vi "Report_path.vi"(8 "error In":errorcluster, 9 "Result":bool) -> (0 "error out":errorcluster, 3 "appended path":path)   [LabVIEW 2021]
panel:
  out "appended path 2":path
  out "path":path
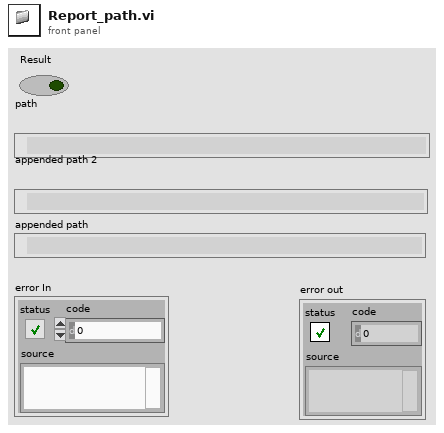
[diagram p1: front panel]
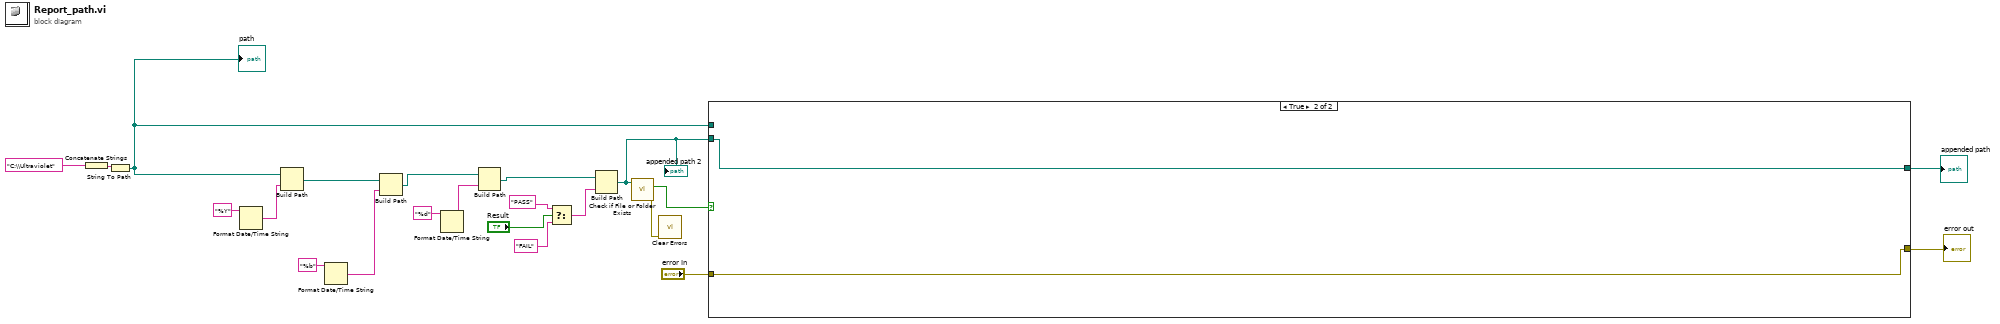
[diagram p0: block diagram]
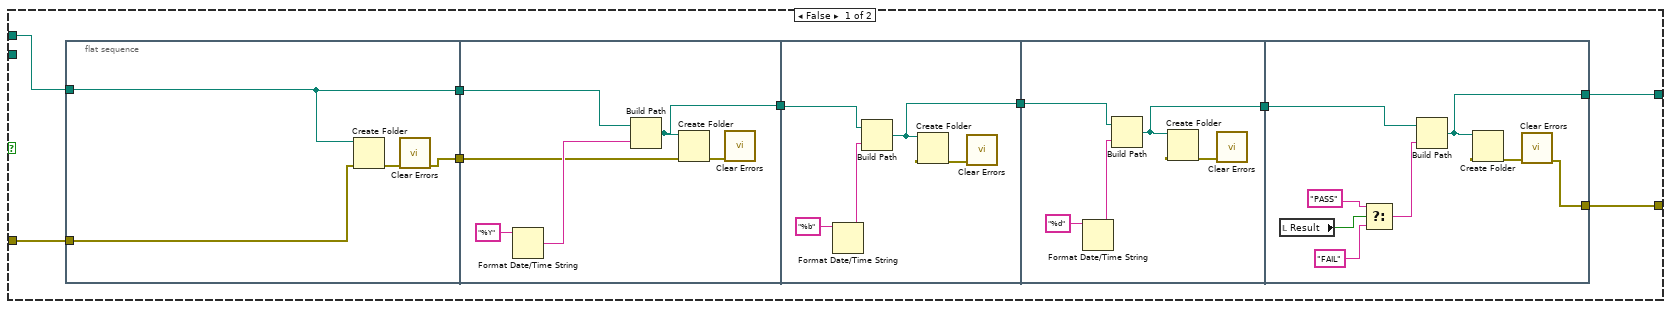
[diagram p2: hidden frame]
diagram:
  n1 = Concatenate Strings("C:\\Ultraviolet" ("string")) -> (w5:string)
  n2 = String To Path(string=w5) -> (path=w3:path)
  "path" <- w3
  n3 = Format Date/Time String(time format string (%c)="%Y") -> (date/time string=w21:string)  [unwired: 2 in]
  n4 = Build Path(base path=w3, name or relative path=w21) -> (appended path=w20:path)
  n5 = Format Date/Time String(time format string (%c)="%b") -> (date/time string=w18:string)  [unwired: 2 in]
  n6 = Build Path(base path=w20, name or relative path=w18) -> (appended path=w15:path)
  n7 = Format Date/Time String(time format string (%c)="%d") -> (date/time string=w17:string)  [unwired: 2 in]
  n8 = Build Path(base path=w15, name or relative path=w17) -> (appended path=w11:path)
  n9 = Select(t="PASS" ("time format string (%c)"), s="Result", f="FAIL" ("time format string (%c)")) -> (s? t:f=w14:string)
  n10 = Build Path(base path=w11, name or relative path=w14) -> (appended path=w8:path)
  "appended path 2" <- w8
  n11 = call <vilib>:"Check if File or Folder Exists.vi"("path"=w8) -> ("error out"=w7:errorcluster, "file or folder exists?"=w6:bool)  [unwired: 8 in, 1 out]
  n12 = call <vilib>:"Clear Errors.vi"("error in (no error)"=w7) -> ()  [unwired: 5 in, 2 out]
  n13 = case shown="True" w6 {
    tunnel: [w27 w61] -> w9
    tunnel: w8 -> [_ w61]
    tunnel: w3 -> [w26 _]
    tunnel: [w25 w60] -> w2
    tunnel: "error In" -> [w24 w60]
    frame False {
      n14 = flat-sequence {
        tunnel: [w34] -> w31
        tunnel: w26 -> [w34]
        tunnel: w24 -> [w33]
        tunnel: [w32] -> w23
        tunnel: [w38] -> w30
        tunnel: w31 -> [w37]
        tunnel: w23 -> [w36]
        tunnel: w30 -> [w44]
        tunnel: [w42] -> w29
        tunnel: w29 -> [w48]
        tunnel: [w47] -> w28
        tunnel: w28 -> [w58]
        tunnel: [w54] -> w27
        tunnel: [w52] -> w25
        frame #0 {
          n15 = Create Folder(path (use dialog)=w34, error in=w33) -> (error out=w35:errorcluster)  [unwired: 1 in, 2 out]
          n16 = call <vilib>:"Clear Errors.vi"("error in (no error)"=w35) -> ("error out"=w32:errorcluster)  [unwired: 5 in, 1 out]
        }
        frame #1 {
          n17 = Format Date/Time String(time format string (%c)="%Y") -> (date/time string=w40:string)  [unwired: 2 in]
          n18 = Build Path(base path=w37, name or relative path=w40) -> (appended path=w38:path)
          n19 = Create Folder(path (use dialog)=w38, error in=w36) -> (error out=w39:errorcluster)  [unwired: 1 in, 2 out]
          n20 = call <vilib>:"Clear Errors.vi"("error in (no error)"=w39) -> ()  [unwired: 5 in, 2 out]
        }
        frame #2 {
          n21 = Format Date/Time String(time format string (%c)="%b") -> (date/time string=w43:string)  [unwired: 2 in]
          n22 = Build Path(base path=w44, name or relative path=w43) -> (appended path=w42:path)
          n23 = Create Folder(path (use dialog)=w42) -> (error out=w46:errorcluster)  [unwired: 2 in, 2 out]
          n24 = call <vilib>:"Clear Errors.vi"("error in (no error)"=w46) -> ()  [unwired: 5 in, 2 out]
        }
        frame #3 {
          n25 = Format Date/Time String(time format string (%c)="%d") -> (date/time string=w51:string)  [unwired: 2 in]
          n26 = Build Path(base path=w48, name or relative path=w51) -> (appended path=w47:path)
          n27 = Create Folder(path (use dialog)=w47) -> (error out=w49:errorcluster)  [unwired: 2 in, 2 out]
          n28 = call <vilib>:"Clear Errors.vi"("error in (no error)"=w49) -> ()  [unwired: 5 in, 2 out]
        }
        frame #4 {
          n29 = local read "Result"() -> (w53:bool)
          n30 = Select(t="PASS" ("time format string (%c)"), s=w53, f="FAIL" ("time format string (%c)")) -> (s? t:f=w55:string)
          n31 = Build Path(base path=w58, name or relative path=w55) -> (appended path=w54:path)
          n32 = Create Folder(path (use dialog)=w54) -> (error out=w59:errorcluster)  [unwired: 2 in, 2 out]
          n33 = call <vilib>:"Clear Errors.vi"("error in (no error)"=w59) -> ("error out"=w52:errorcluster)  [unwired: 5 in, 1 out]
        }
      }
    }
    frame True {
    }
  }
  "appended path" <- w9
  "error out" <- w2
